vi "Rename python module to generic name.vi"(11 "Test Case In":refnum<class "Runner Unit Test - Prepare Project.lvclass">) -> (0 "error out":errorcluster, 3 "Test Case Out":refnum<class "Runner Unit Test - Prepare Project.lvclass">)   [LabVIEW 2026, in "Runner Unit Test - Prepare Project.lvclass"]
uses:
  Runner Unit Test - Prepare Project.lvclass
  C:/Program Files/National Instruments/LabVIEW 2026/vi.lib/Astemes/LUnit/Test Case.lvclass
  Actors/Runner/Runner/Runner.lvclass
  Interfaces/IRunner/IRunner/Interfaces--cluster.ctl
  Interfaces/IProject Manager/IProject Manager.lvclass
  Interfaces/IFile Manager/IFile Manager.lvclass
  Interfaces/IPython Caller/IPython Caller.lvclass
  Interfaces/IElement Manager/IElement Manager.lvclass
  Interfaces/ILV File Creator/ILV File Creator.lvclass
  Interfaces/IHash Whitelist Handler/IHash Whitelist Handler.lvclass
  Actors/Mock Logger/Mock Logger/Mock Logger.lvclass
  C:/Program Files/National Instruments/LabVIEW 2026/vi.lib/ActorFramework/Actor/Actor.lvclass
  <vilib>/ActorFramework/Message Enqueuer/Message Enqueuer.lvclass/Message Enqueuer.ctl
  <vilib>/ActorFramework/Message Enqueuer/Enqueue.vi
  Mocks/Mock IFile Manager/Mock IFile Manager.lvclass
  C:/Program Files/National Instruments/LabVIEW 2026/vi.lib/Astemes/LMock/Mock.lvclass
  C:/Users/juanj/Documents/hasbun_wood_engineering/github/py2vi/labview/Interfaces/IFile Manager/IFile Manager.lvclass
  <vilib>/ActorFramework/Stop Msg/Stop Msg.lvclass
  C:/Program Files/National Instruments/LabVIEW 2026/vi.lib/ActorFramework/Message/Message.lvclass
  <vilib>/Astemes/LMock/One Identical Inputs.vi
  <vilib>/ActorFramework/Message Priority Queue/Priority Enqueue.vi
  C:/Users/juanj/Documents/hasbun_wood_engineering/github/py2vi/labview/Mocks/Mock IFile Manager/Mock IFile Manager.lvclass
  Interfaces/IRunner/IRunner/IRunner.lvclass
  <vilib>/ActorFramework/Actor/Actor.lvclass
  <vilib>/Astemes/LMock/LMock Verifier.lvclass
  <vilib>/Astemes/LMock/LMock.lvlib
  <vilib>/Astemes/LMock/LMock One.lvlib
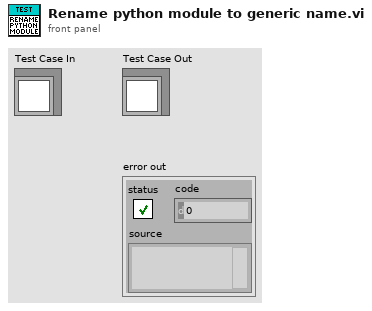
[diagram p1: front panel]
types:
  T1 = typedef "IRunner.lvlib/IRunner.lvclass/Interfaces--cluster.ctl" = cluster{"IProject Manager":refnum<class "IProject Manager.lvclass">, "IFile Manager":refnum<class "IFile Manager.lvclass">, "IPython Caller":refnum<class "IPython Caller.lvclass">, "IElement Manager":refnum<class "IElement Manager.lvclass">, "ILV File Creator":refnum<class "ILV File Creator.lvclass">, "IHash Whitelist Handler":refnum<class "IHash Whitelist Handler.lvclass">}
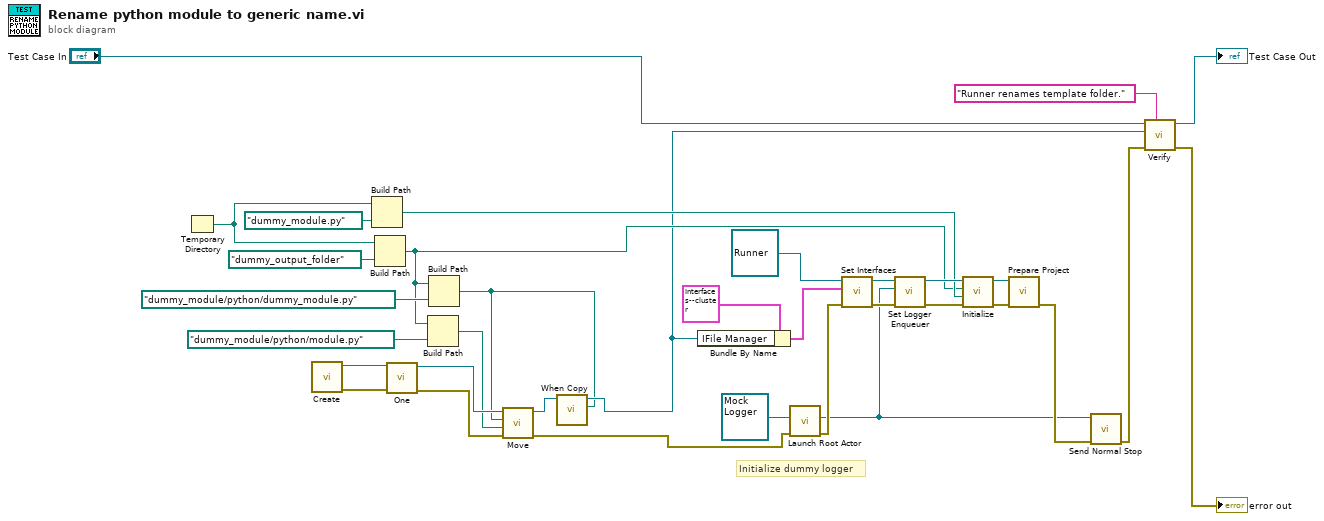
[diagram p0: block diagram]
diagram:
  # "Initialize dummy logger"
  n1 = Temporary Directory() -> (w8:path)
  n2 = call "Create.vi"() -> ("error out"=w33:errorcluster, "Mock Class Generator out"=w20:refnum<class "Mock IFile Manager.lvclass">)  [unwired: 10 in]
  n3 = Build Path(base path=w8, name or relative path=path "dummy_module.py") -> (appended path=w12:path)
  n4 = Build Path(base path=w8, name or relative path=path "dummy_output_folder") -> (appended path=w4:path)
  n5 = call-poly <vilib>:"One.vi"("error in (no error)"=w33, "Mock in"=w20) -> ("error out"=w26:errorcluster, "Mock out"=w9:refnum<class "Mock IFile Manager.lvclass">)  [unwired: 8 in]
  n6 = Build Path(base path=w4, name or relative path=path "dummy_module/python/module.py") -> (appended path=w6:path)
  n7 = Build Path(base path=w4, name or relative path=path "dummy_module/python/dummy_module.py") -> (appended path=w1:path)
  n8 = call-dynamic "Move.vi"("error in"=w26, "Target"=w6, "Source"=w1, "IFile Manager in"=w9) -> ("error out"=w25:errorcluster, "IFile Manager out"=w3:refnum<class "Mock IFile Manager.lvclass">)  [unwired: 6 in]
  n9 = call "When Copy.vi"("New Path"=w1, "IFile Manager in"=w3) -> ("IFile Manager out"=w2:refnum<class "Mock IFile Manager.lvclass">)  [unwired: 9 in]
  n10 = Bundle By Name(cluster=T1 {"IProject Manager"=refnum, "IFile Manager"=refnum, "IPython Caller"=refnum, "IElement Manager"=refnum, "ILV File Creator"=refnum, "IHash Whitelist Handler"=refnum} ("Interfaces"), "IFile Manager"=w2) -> (w21:T1)
  n11 = call <vilib>:"Launch Root Actor.vi"("error in (no error)"=w25, "Actor"=refnum<class "Mock Logger.lvclass"> refnum ("Mock Logger.lvlib:Mock Logger.lvclass")) -> ("error out"=w32:errorcluster, "Actor's Enqueuer"=w18:refnum<class "Message Enqueuer.lvclass">)  [unwired: 8 in]
  n12 = call-dynamic "Set Interfaces.vi"("error in"=w32, "Interfaces"=w21, "Runner in"=refnum<class "Runner.lvclass"> refnum ("Runner.lvlib:Runner.lvclass")) -> ("error out"=w34:errorcluster, "Runner out"=w23:refnum<class "Runner.lvclass">)  [unwired: 7 in]
  n13 = call-dynamic "Set Logger Enqueuer.vi"("error in"=w34, "Logger"=w18, "Runner in"=w23) -> ("error out"=w29:errorcluster, "Runner out"=w15:refnum<class "Runner.lvclass">)  [unwired: 7 in]
  n14 = call-dynamic "Initialize.vi"("error in"=w29, "Python Module"=w12, "Output Folder"=w4, "G-CLI Runner in"=w15) -> ("error out"=w28:errorcluster, "G-CLI Runner out"=w14:refnum<class "Runner.lvclass">)  [unwired: 6 in]
  n15 = call-dynamic "Prepare Project.vi"("error in"=w28, "G-CLI Runner in"=w14) -> ("error out"=w31:errorcluster)  [unwired: 8 in, 1 out]
  n16 = call <vilib>:"Send Normal Stop.vi"("error in (no error)"=w31, "Message Enqueuer"=w18) -> ("error out"=w30:errorcluster)  [unwired: 9 in]
  n17 = call <vilib>:"Verify.vi"("Description"="Runner renames template folder.", "error in (no error)"=w30, "Mock"=w2, "LUnit Test Case In"="Test Case In") -> ("error out"=→"error out":errorcluster, "LUnit Test Case Out"=→"Test Case Out":refnum<class "Runner Unit Test - Prepare Project.lvclass">)  [unwired: 6 in]
